vi "Parse_procotol_sub.vi"(8 "Frame":string, 9 "ID_index":i32[](array[numeric]), 10 "Name_signal":string[](array[string]), 11 "Procotol":string[][](array[string])) -> (1 "Mean":string[](array[string]), 2 "Valid/Matched?":bool[](array[boolean]), 3 "ARR_numb":string[](array[string]))   [LabVIEW 2025, in "Procotol_class.lvclass"]
uses:
  Procotol_class.lvclass
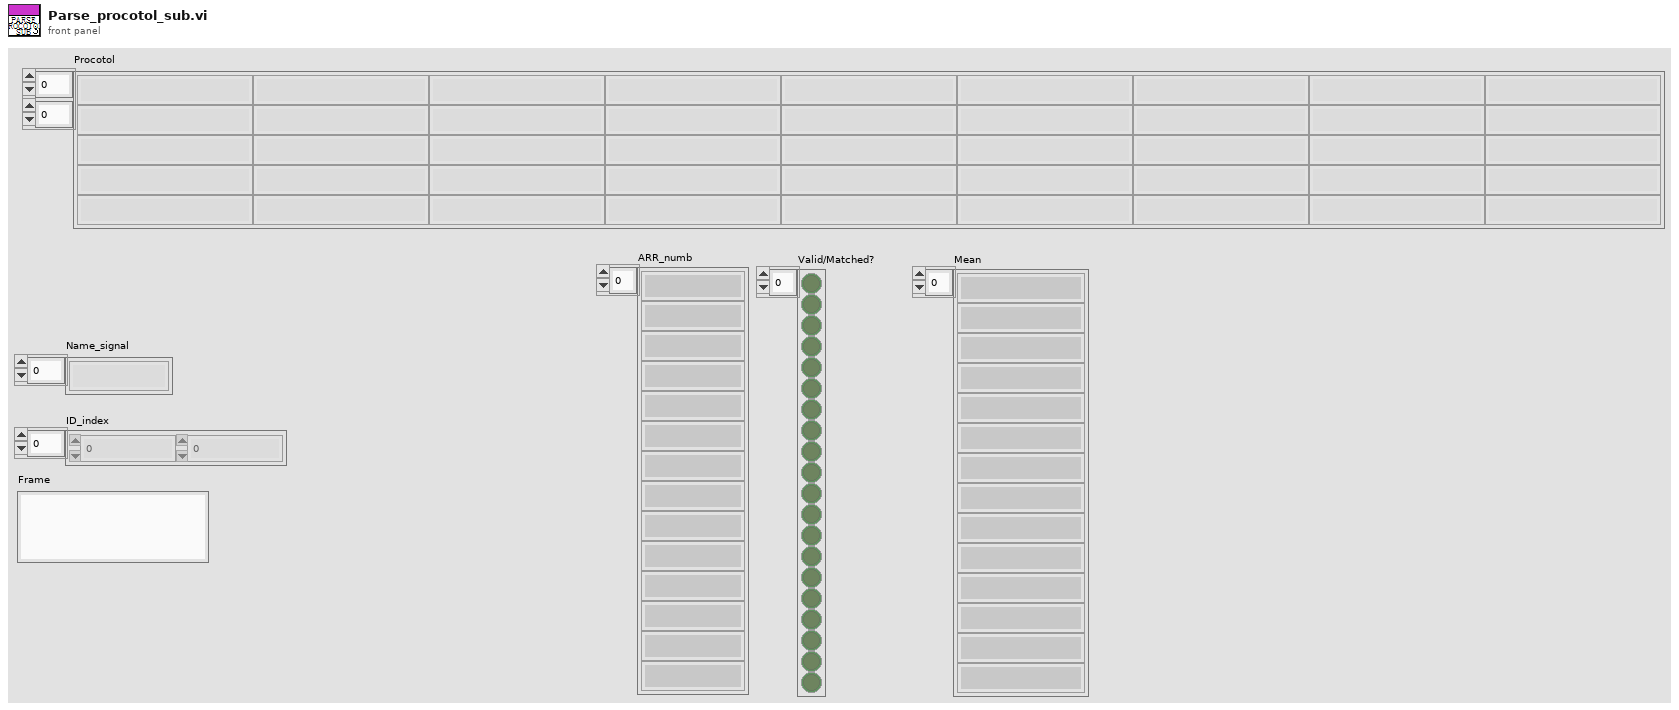
[diagram p1: front panel]
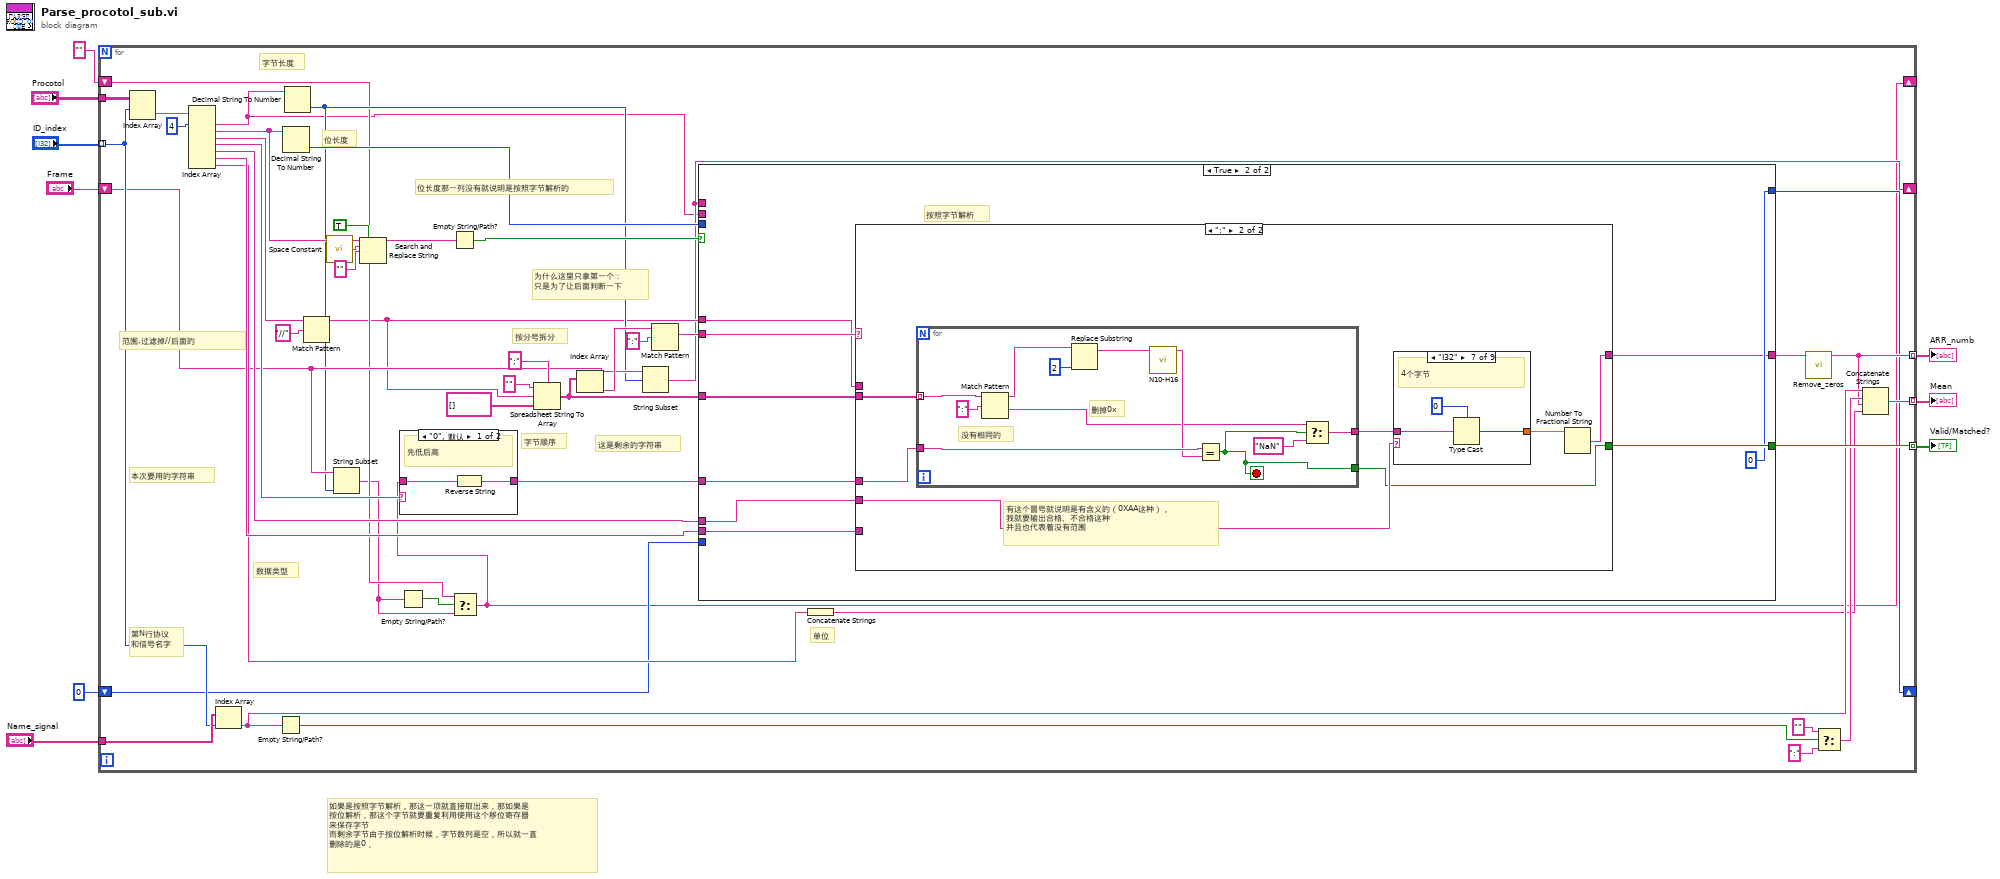
[diagram p0: block diagram]
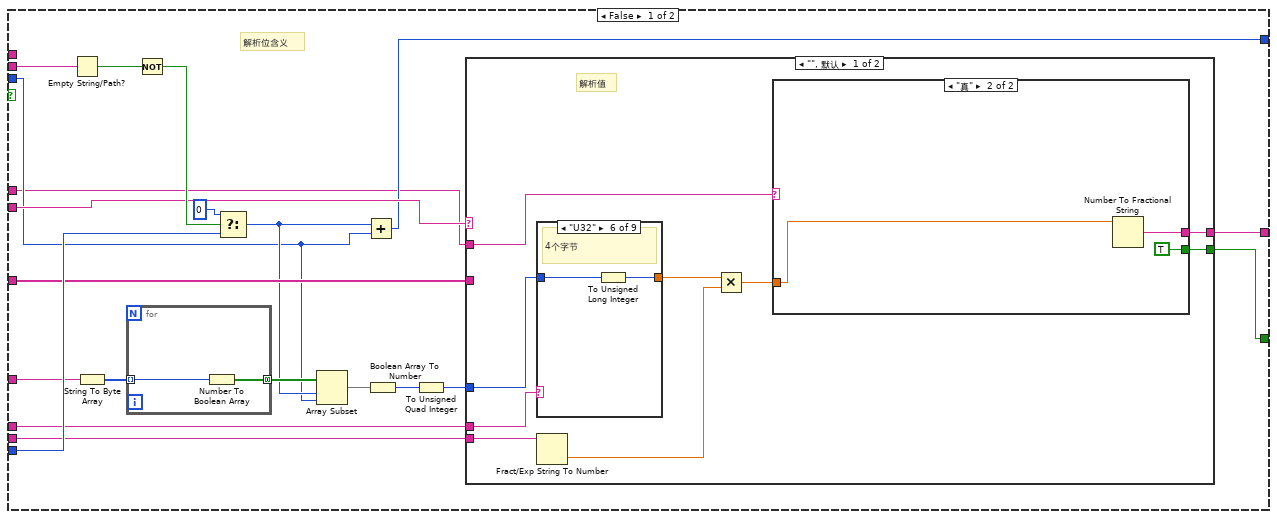
[diagram p2: hidden frame]
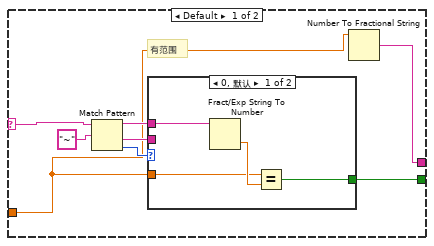
[diagram p3: hidden frame]
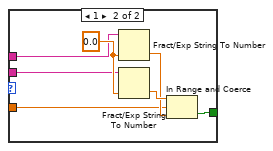
[diagram p4: hidden frame]
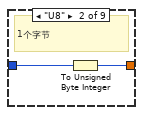
[diagram p6: hidden frame]
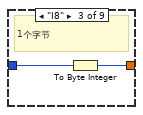
[diagram p7: hidden frame]
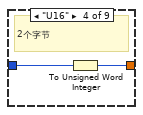
[diagram p8: hidden frame]
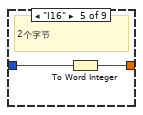
[diagram p9: hidden frame]
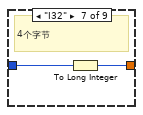
[diagram p10: hidden frame]
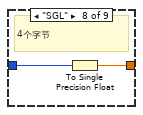
[diagram p11: hidden frame]
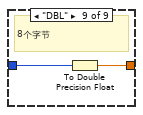
[diagram p12: hidden frame]
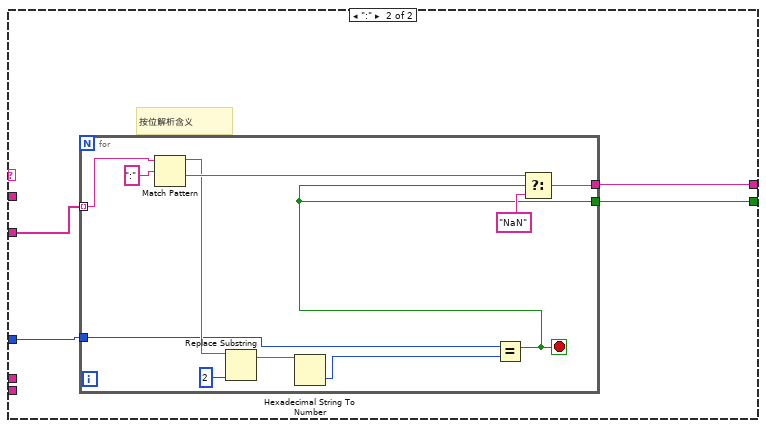
[diagram p13: hidden frame]
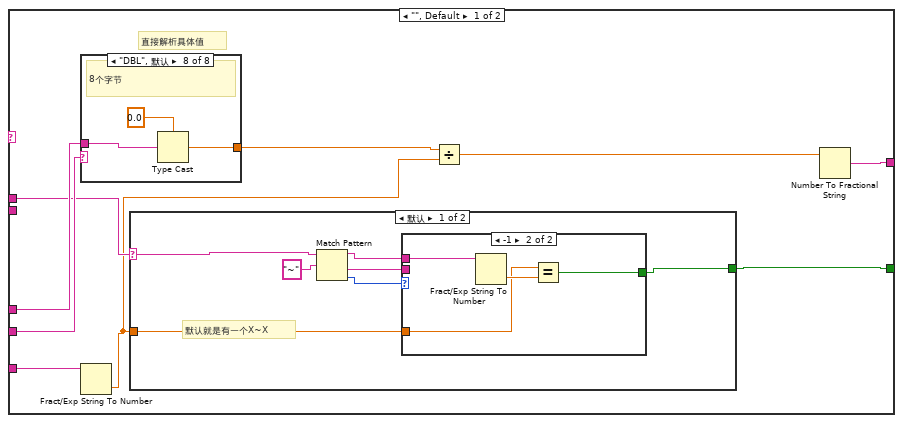
[diagram p14: hidden frame]
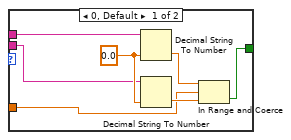
[diagram p15: hidden frame]
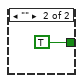
[diagram p16: hidden frame]
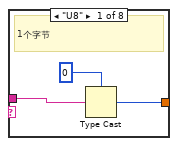
[diagram p17: hidden frame]
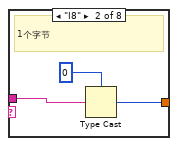
[diagram p18: hidden frame]
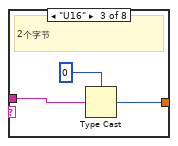
[diagram p19: hidden frame]
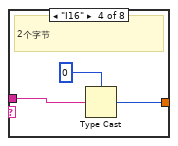
[diagram p20: hidden frame]
diagram:
  # "如果是按照字节解析，那这一项就直接取出来，那如果是\n按位解析，那这个字节就要重复利用使用这个移位寄存器\n来保存字节\n而剩余字节由于按位解析时候，字节数列是空，所以就一直\n删除的是0，"
  n1 = for {
    tunnel: "Procotol" -> [w56]
    tunnel: "ID_index" -> [w54] mode=indexing
    tunnel: "Name_signal" -> [w55]
    shift-right: [w13] -> _
    shift-left: "Frame" -> [w32]
    shift-right: [w10] -> _
    shift-left: "" ("原始帧") -> [w29]
    tunnel: [w18] -> w4 mode=indexing
    tunnel: [w24] -> w3 mode=indexing
    tunnel: [w16] -> w2 mode=indexing
    shift-right: [w14] -> _
    shift-left: 0 -> [w15]
    # "位长度那一列没有就说明是按照字节解析的"
    # "为什么这里只拿第一个：\n只是为了让后面判断一下"
    # "本次要用的字符串"
    # "这是剩余的字符串"
    # "单位"
    # "按分号拆分"
    # "数据类型"
    # "字节顺序"
    # "范围,过滤掉//后面的"
    # "位长度"
    # "字节长度"
    # "第N行协议\n和信号名字"
    n2 = Index Array(array=w56, index (row)=w54) -> (element=w53:string[])  [unwired: 1 in]
    n3 = Index Array(array=w53, index #1=4 ("索引")) -> (element #1=w12:string, element #2=w36:string, element #3=w50:string, element #4=w49:string, element #5=w48:string, element #6=w47:string, element #7=w33:string)  [unwired: 6 in]
    n4 = Index Array(array=w55, index=w54) -> (element=w20:string)
    n5 = Empty String/Path?(string/path=w20) -> (empty?=w22:bool)
    n6 = Decimal String To Number(string=w36) -> (number=w34:i32)  [unwired: 2 in, 1 out]
    n7 = Decimal String To Number(string=w12) -> (number=w31:i32)  [unwired: 2 in, 1 out]
    n8 = Match Pattern(string=w50, regular expression="//" ("正则表达式")) -> (before substring=w27:string)  [unwired: 1 in, 3 out]
    n9 = call <vilib>:"Space Constant.vi"() -> ("String"=w40:string)
    n10 = String Subset(string=w32, length (rest)=w31) -> (substring=w28:string)  [unwired: 1 in]
    n11 = Search and Replace String(replace all?=TRUE ("替换全部？(F)"), input string=w36, search string=w40, replace string="" ("替换字符串(\"\")")) -> (result string=w37:string)  [unwired: 4 in, 3 out]
    n12 = Empty String/Path?(string/path=w28) -> (empty?=w30:bool)
    n13 = Empty String/Path?(string/path=w37) -> (empty?=w35:bool)
    n14 = Select(t=w29, s=w30, f=w28) -> (s? t:f=w10:string)
    n15 = case shown="\"0\", 默认" w49 {
      tunnel: [w247 w248] -> w25
      tunnel: w10 -> [w246 w248]
      frame "0", Default {
        # "先低后高"
        n16 = Reverse String(1:w246) -> (0:w247:string)
      }
      frame "1" {
        # "先高后低"
      }
    }
    n17 = Spreadsheet String To Array(delimiter (Tab)=";" ("分隔符(Tab)"), format string="" ("格式字符串"), spreadsheet string=w27, array type (2D Dbl)=string[] [] ("数组")) -> (array=w26:string[])
    n18 = Index Array(array=w26) -> (element=w43:string)  [unwired: 1 in]
    n19 = String Subset(string=w32, offset (0)=w31) -> (substring=w13:string)  [unwired: 1 in]
    n20 = Match Pattern(string=w43, regular expression=":") -> (match substring=w41:string)  [unwired: 1 in, 3 out]
    n21 = case shown="True" w35 {
      tunnel: w41 -> [w67 w151]
      tunnel: w34 -> [w62 _]
      tunnel: w48 -> [w60 w150]
      tunnel: w47 -> [w59 w149]
      tunnel: w27 -> [w58 w148]
      tunnel: w26 -> [w66 w147]
      tunnel: w25 -> [w68 w146]
      tunnel: [w64 w145] -> w24
      tunnel: w15 -> [w73 _]
      tunnel: [w61 0] -> w14
      tunnel: w13 -> [_ _]
      tunnel: w12 -> [w74 _]
      tunnel: [w57 w143] -> w11
      frame False {
        # "解析位含义"
        n22 = Empty String/Path?(string/path=w74) -> (empty?=w76:bool)
        n23 = String To Byte Array(string=w68) -> (unsigned byte array=w72:u8[])
        n24 = for {
          tunnel: w72 -> [w142] mode=indexing
          tunnel: [w141] -> w69 mode=concatenating
          n25 = Number To Boolean Array(number=w142) -> (Boolean array=w141:bool[])
        }
        n26 = Not(x=w76) -> (.not. x?=w75:bool)
        n27 = Select(t=0, s=w75, f=w73) -> (s? t:f=w63:i32)
        n28 = Array Subset(array=w69, index=w63, length=w62) -> (w71:bool[])
        n29 = Add(x=w63, y=w62) -> (x+y=w61:i32)
        n30 = Boolean Array To Number(Boolean array=w71) -> (number=w70:u32)
        n31 = To Unsigned Quad Integer(1:w70) -> (0:w65:u64)
        n32 = case shown="\"\", 默认" w67 {
          tunnel: w66 -> [_ w128]
          tunnel: w65 -> [w85 w129]
          tunnel: [w79 w127] -> w64
          tunnel: w60 -> [w86 _]
          tunnel: w59 -> [w82 _]
          tunnel: w58 -> [w81 _]
          tunnel: [w78 w126] -> w57
          frame "", Default {
            # "解析值"
            n33 = case shown="\"U32\"" w86 {
              tunnel: w85 -> [w109 w111 w113 w115 w117 w119 w121 w123 w125]
              tunnel: [w109 w110 w112 w114 w116 w118 w120 w122 w124] -> w84
              frame "", Default {
                # "数据类型"
              }
              frame "U8" {
                # "1个字节"
                n34 = To Unsigned Byte Integer(number=w111) -> (unsigned 8bit integer=w110:u8)
              }
              frame "I8" {
                # "1个字节"
                n35 = To Byte Integer(number=w113) -> (8bit integer=w112:i8)
              }
              frame "U16" {
                # "2个字节"
                n36 = To Unsigned Word Integer(number=w115) -> (unsigned 16bit integer=w114:u16)
              }
              frame "I16" {
                # "2个字节"
                n37 = To Word Integer(number=w117) -> (16bit integer=w116:i16)
              }
              frame "U32" {
                # "4个字节"
                n38 = To Unsigned Long Integer(number=w119) -> (unsigned 32bit integer=w118:u32)
              }
              frame "I32" {
                # "4个字节"
                n39 = To Long Integer(number=w121) -> (32bit integer=w120:i32)
              }
              frame "SGL" {
                # "4个字节"
                n40 = To Single Precision Float(number=w123) -> (single precision float=w122:sgl)
              }
              frame "DBL" {
                # "8个字节"
                n41 = To Double Precision Float(number=w125) -> (double precision float=w124:dbl)
              }
            }
            n42 = Fract/Exp String To Number(string=w82) -> (number=w83:dbl)  [unwired: 3 in, 1 out]
            n43 = Multiply(x=w84, y=w83) -> (x*y=w80:dbl)
            n44 = case shown="\"真\"" w81 {
              selector: w81 -> [w93 _]
              tunnel: w80 -> [w88 w107]
              tunnel: [w89 TRUE] -> w79
              tunnel: [w87 w108] -> w78
              frame Default {
                # "有范围"
                n45 = Match Pattern(string=w93, regular expression="~" ("正则表达式")) -> (before substring=w92:string, after substring=w90:string, offset past match=w91:i32)  [unwired: 1 in, 1 out]
                n46 = case shown="0, 默认" w91 {
                  tunnel: w92 -> [w97 w102]
                  tunnel: w90 -> [_ w101]
                  tunnel: w88 -> [w96 w100]
                  tunnel: [w95 w99] -> w89
                  frame 0, Default {
                    n47 = Fract/Exp String To Number(string=w97) -> (number=w98:dbl)  [unwired: 3 in, 1 out]
                    n48 = Equal?(x=w96, y=w98) -> (x = y?=w95:bool)
                  }
                  frame 1 {
                    w104 = 0.0 ("默认(0 I32)")
                    n49 = Fract/Exp String To Number(string=w102, default (0 dbl)=w104) -> (number=w103:dbl)  [unwired: 2 in, 1 out]
                    n50 = Fract/Exp String To Number(string=w101, default (0 dbl)=w104) -> (number=w105:dbl)  [unwired: 2 in, 1 out]
                    n51 = In Range and Coerce(upper limit=w105, x=w100, lower limit=w103) -> (In Range?=w99:bool)  [unwired: 1 out]
                  }
                }
                n52 = Number To Fractional String(number=w88) -> (F-format string=w87:string)  [unwired: 3 in]
              }
              frame "真" {
                n53 = Number To Fractional String(number=w107) -> (F-format string=w108:string)  [unwired: 3 in]
              }
            }
          }
          frame ":" {
            # "按位解析含义"
            n54 = for {
              tunnel: w128 -> [w139] mode=indexing
              tunnel: [w136] -> w126
              tunnel: [w135] -> w127
              tunnel: w129 -> [w132]
              stop <- w135 stop-if-true
              n55 = Match Pattern(string=w139, regular expression=":" ("正则表达式")) -> (before substring=w133:string, after substring=w137:string)  [unwired: 1 in, 2 out]
              n56 = Replace Substring(2:2 ("长度（子字符串长度）"), 5:w133) -> (1:w131:string)  [unwired: 2 in, 1 out]
              n57 = Hexadecimal String To Number(string=w131) -> (number=w130:u32)  [unwired: 2 in, 1 out]
              n58 = Equal?(x=w132, y=w130) -> (x = y?=w135:bool)
              n59 = Select(t=w137, s=w135, f="NaN") -> (s? t:f=w136:string)
            }
          }
        }
      }
      frame True {
        # "按照字节解析"
        n60 = case shown="\":\"" w151 {
          tunnel: w150 -> [w159 w208]
          tunnel: w149 -> [w158 _]
          tunnel: w148 -> [w157 _]
          tunnel: w147 -> [_ w210]
          tunnel: w146 -> [w160 w209]
          tunnel: [w155 w206] -> w143
          tunnel: [w156 w205] -> w145
          frame "", Default {
            # "直接解析具体值"
            n61 = case shown="\"DBL\", 默认" w159 {
              tunnel: w160 -> [w182 w185 w188 w191 w192 w195 w200 w203]
              tunnel: [w180 w183 w186 w189 w193 w196 w198 w201] -> w154
              frame "U8" {
                # "1个字节"
                n62 = Type Cast(type=u8 0, x=w182) -> (*(type *) &x=w180:u8)
              }
              frame "I8" {
                # "1个字节"
                n63 = Type Cast(type=i8 0, x=w185) -> (*(type *) &x=w183:i8)
              }
              frame "U16" {
                # "2个字节"
                n64 = Type Cast(type=u16 0, x=w188) -> (*(type *) &x=w186:u16)
              }
              frame "I16" {
                # "2个字节"
                n65 = Type Cast(type=i16 0, x=w191) -> (*(type *) &x=w189:i16)
              }
              frame "U32" {
                # "4个字节"
                n66 = Type Cast(type=u32 0, x=w192) -> (*(type *) &x=w193:u32)
              }
              frame "I32" {
                # "4个字节"
                n67 = Type Cast(type=0, x=w195) -> (*(type *) &x=w196:i32)
              }
              frame "SGL" {
                # "4个字节"
                n68 = Type Cast(type=sgl 0.0, x=w200) -> (*(type *) &x=w198:sgl)
              }
              frame "DBL", Default {
                # "8个字节"
                n69 = Type Cast(type=0.0, x=w203) -> (*(type *) &x=w201:dbl)
              }
            }
            n70 = Fract/Exp String To Number(string=w158) -> (number=w153:dbl)  [unwired: 3 in, 1 out]
            n71 = case shown="默认" w157 {
              selector: w157 -> [w166 _]
              tunnel: w153 -> [w165 _]
              tunnel: [w162 TRUE] -> w156
              frame Default {
                # "默认就是有一个X~X"
                n72 = Match Pattern(string=w166, regular expression="~" ("正则表达式")) -> (before substring=w164:string, after substring=w163:string, offset past match=w161:i32)  [unwired: 1 in, 1 out]
                n73 = case shown="-1" w161 {
                  tunnel: w165 -> [w171 w176]
                  tunnel: w164 -> [w170 w177]
                  tunnel: w163 -> [w169 _]
                  tunnel: [w168 w175] -> w162
                  frame 0, Default {
                    w173 = 0.0 ("默认(0 I32)")
                    n74 = Decimal String To Number(string=w170, default (0L)=w173) -> (number=w174:dbl)  [unwired: 1 in, 1 out]
                    n75 = Decimal String To Number(string=w169, default (0L)=w173) -> (number=w172:dbl)  [unwired: 1 in, 1 out]
                    n76 = In Range and Coerce(upper limit=w174, x=w171, lower limit=w172) -> (In Range?=w168:bool)  [unwired: 1 out]
                  }
                  frame -1 {
                    n77 = Fract/Exp String To Number(string=w177) -> (number=w178:dbl)  [unwired: 3 in, 1 out]
                    n78 = Equal?(x=w176, y=w178) -> (x = y?=w175:bool)
                  }
                }
              }
              frame "" {
              }
            }
            n79 = Divide(x=w154, y=w153) -> (x/y=w152:dbl)
            n80 = Number To Fractional String(number=w152) -> (F-format string=w155:string)  [unwired: 3 in]
          }
          frame ":" {
            # "有这个冒号就说明是有含义的（0XAA这种），\n我就要输出合格、不合格这种\n并且也代表着没有范围"
            n81 = for {
              tunnel: w210 -> [w242] mode=indexing
              tunnel: w209 -> [w240]
              tunnel: [w237] -> w205
              tunnel: [w235] -> w204
              stop <- w237 stop-if-true
              # "没有相同的"
              # "删掉0x"
              n82 = Match Pattern(string=w242, regular expression=":" ("正则表达式")) -> (before substring=w245:string, after substring=w236:string)  [unwired: 1 in, 2 out]
              n83 = Replace Substring(2:2 ("长度（子字符串长度）"), 5:w245) -> (1:w241:string)  [unwired: 2 in, 1 out]
              n84 = call "N10-H16.vi"("Str_10"=w241) -> ("Str_16"=w239:string)  [unwired: 10 in]
              n85 = Equal?(x=w240, y=w239) -> (x = y?=w237:bool)
              n86 = Select(t=w236, s=w237, f="NaN") -> (s? t:f=w235:string)
            }
            n87 = case shown="\"I32\"" w208 {
              tunnel: [_ w212 w215 w218 w221 w224 w227 w230 w233] -> w207
              tunnel: w204 -> [_ w211 w214 w217 w220 w223 w226 w229 w232]
              frame "", Default {
                # "数据类型"
              }
              frame "U8" {
                # "1个字节"
                n88 = Type Cast(type=u8 0, x=w211) -> (*(type *) &x=w212:u8)
              }
              frame "I8" {
                # "1个字节"
                n89 = Type Cast(type=i8 0, x=w214) -> (*(type *) &x=w215:i8)
              }
              frame "U16" {
                # "2个字节"
                n90 = Type Cast(type=u16 0, x=w217) -> (*(type *) &x=w218:u16)
              }
              frame "I16" {
                # "2个字节"
                n91 = Type Cast(type=i16 0, x=w220) -> (*(type *) &x=w221:i16)
              }
              frame "U32" {
                # "4个字节"
                n92 = Type Cast(type=u32 0, x=w223) -> (*(type *) &x=w224:u32)
              }
              frame "I32" {
                # "4个字节"
                n93 = Type Cast(type=0, x=w226) -> (*(type *) &x=w227:i32)
              }
              frame "SGL" {
                # "4个字节"
                n94 = Type Cast(type=sgl 0.0, x=w229) -> (*(type *) &x=w230:sgl)
              }
              frame "DBL" {
                # "8个字节"
                n95 = Type Cast(type=0.0, x=w232) -> (*(type *) &x=w233:dbl)
              }
            }
            n96 = Number To Fractional String(number=w207) -> (F-format string=w206:string)  [unwired: 3 in]
          }
        }
      }
    }
    n97 = Concatenate Strings(w33) -> (w17:string)
    n98 = call "Remove_zeros.vi"("Float_char"=w11) -> ("float_adaptive"=w18:string)  [unwired: 10 in]
    n99 = Select(t="", s=w22, f=":") -> (s? t:f=w19:string)
    n100 = Concatenate Strings(w20, w19, w18, w17) -> (w16:string)
  }
  "ARR_numb" <- w4
  "Valid/Matched?" <- w3
  "Mean" <- w2
